vi "PicoScope2000AdvancedTriggerSettings.vi"(0 "handle in":i16, 2 "Pulse Width Qualifier Conditions":T4 {"Condition Logic" items=["AND", "OR", "XOR"]}, 3 "Pulse Width Qualifier Settings":T3 {"Pulse Width Type" items=["None", "Less Than", "Greater Than", "In Range", "Out of Range"]; "Direction" items=["Rising", "Falling"]}, 5 "error in":errorcluster, 6 "Trigger Conditions":T1 {"PWQ" items=["Don't Care", "True", "False"]; "Ext" items=["Don't Care", "True", "False"]; "Channel D" items=["Don't Care", "True", "False"]; "Channel C" items=["Don't Care", "True", "False"]; "Channel B" items=["Don't Care", "True", "False"]; "Channel A" items=["Don't Care", "True", "False"]; "Condition Logic" items=["AND", "OR", "XOR"]}, 7 "Auto Trigger (ms)":i32, 8 "Channel A Trigger Properties":T2 {"Direction" items=["Above / Inside", "Below / Outside", "Rising / Enter", "Falling / Exit", "Rising or Falling / Enter or Exit", "Above Lower", "Below Lower", "Rising Lower", "Falling Lower", "Positive Runt", "Negative Runt"]; "Threshold Mode" items=["Level", "Window"]}, 9 "Trigger Delay":u32, 10 "Channel B Trigger Properties":T2 {"Direction" items=["Above / Inside", "Below / Outside", "Rising / Enter", "Falling / Exit", "Rising or Falling / Enter or Exit", "Above Lower", "Below Lower", "Rising Lower", "Falling Lower", "Positive Runt", "Negative Runt"]; "Threshold Mode" items=["Level", "Window"]}, 11 "preTriggerDelay":sgl, 12 "Ext. Trigger Properties":T2 {"Direction" items=["Above / Inside", "Below / Outside", "Rising / Enter", "Falling / Exit", "Rising or Falling / Enter or Exit", "Above Lower", "Below Lower", "Rising Lower", "Falling Lower", "Positive Runt", "Negative Runt"]; "Threshold Mode" items=["Level", "Window"]}) -> (14 "handle out":i16, 19 "error out":errorcluster)   [LabVIEW 2009]
doc: "This VI is an interface for the advanced trigger features of the oscilloscope (a simple trigger can be set using PicoScope2000Settings.vi, in which case it is not necessary to use this VI)."
uses:
  ps2000.dll
panel:
  in  "Channel D Trigger Properties":T2 {"Direction" items=["Above / Inside", "Below / Outside", "Rising / Enter", "Falling / Exit", "Rising or Falling / Enter or Exit", "Above Lower", "Below Lower", "Rising Lower", "Falling Lower", "Positive Runt", "Negative Runt"]; "Threshold Mode" items=["Level", "Window"]}
  in  "Channel C Trigger Properties":T2 {"Direction" items=["Above / Inside", "Below / Outside", "Rising / Enter", "Falling / Exit", "Rising or Falling / Enter or Exit", "Above Lower", "Below Lower", "Rising Lower", "Falling Lower", "Positive Runt", "Negative Runt"]; "Threshold Mode" items=["Level", "Window"]}
  # "For Condition Logic Suggested settings;\nFor AND, XOR logic-(parallel triggers)\nUse level-type triggers (Level or Inside/outside Window Triggers)\n\nFor OR logic- (single channel)\nUse edge types (e.g. rising, falling, entering window)"
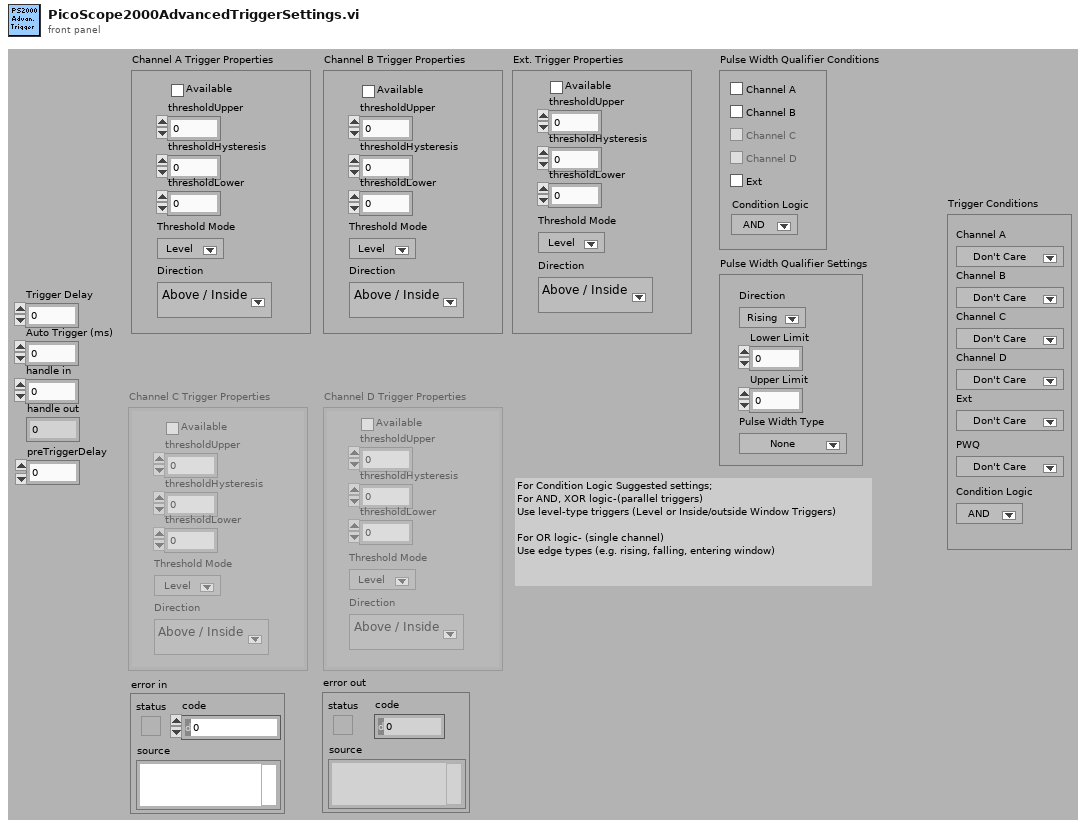
[diagram p1: front panel]
types:
  T1 = cluster{"Channel A":u16, "Channel B":u16, "Channel C":u16, "Channel D":u16, "Ext":u16, "PWQ":u16, "Condition Logic":u16}
  T2 = cluster{"thresholdUpper":i16, "thresholdHysteresis":u16, "thresholdLower":i16, "Threshold Mode":i32, "Direction":i32, "Available":bool}
  T3 = cluster{"Direction":u32, "Lower Limit":u32, "Upper Limit":u32, "Pulse Width Type":u32}
  T4 = cluster{"Channel A":bool, "Channel B":bool, "Channel C":bool, "Channel D":bool, "Condition Logic":u16, "Ext":bool}
  T5 = cluster{"thresholdUpper":i16, "thresholdHysteresis":u16, "thresholdLower":i16, "Threshold Mode":i32, "Direction":i32, "Available":bool}[]
  T6 = cluster{"[0]":u32, "[1]":u32, "[2]":u32, "[3]":u32, "[4]":u32, "[5]":u32, "[6]":u32, "[7]":u32, "[8]":u32}
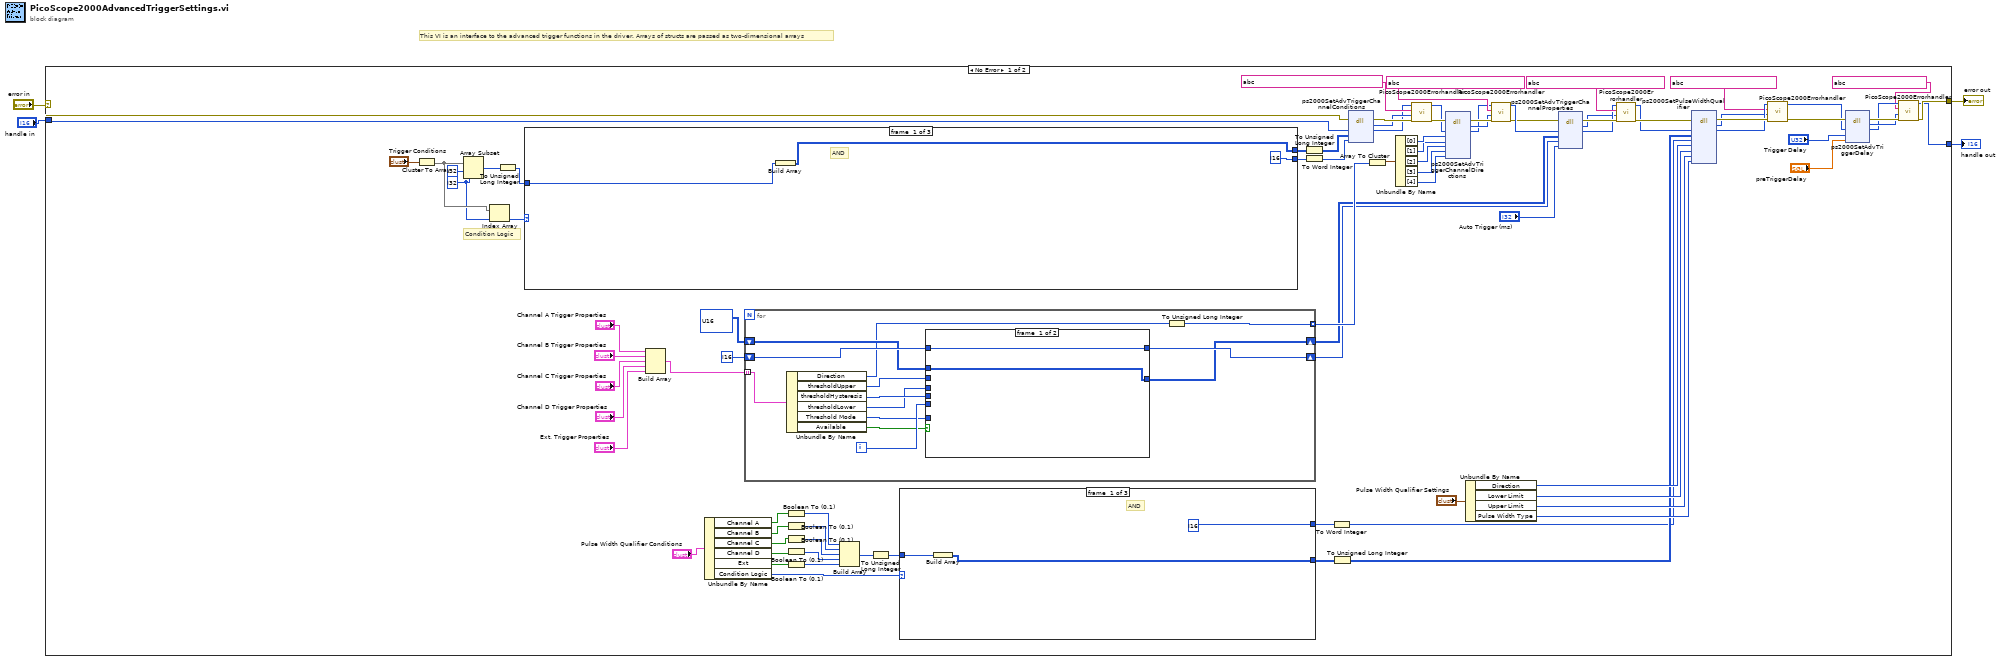
[diagram p0: block diagram]
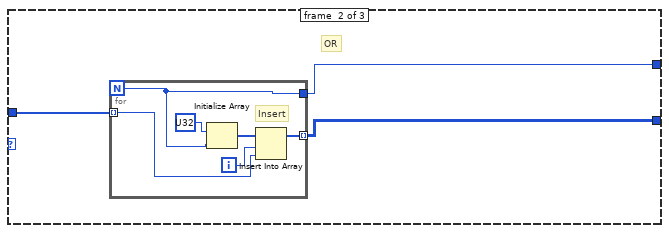
[diagram p2: hidden frame]
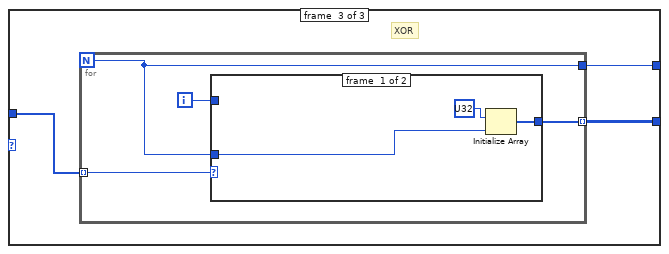
[diagram p3: hidden frame]
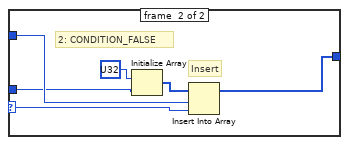
[diagram p4: hidden frame]
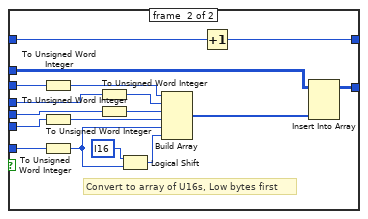
[diagram p5: hidden frame]
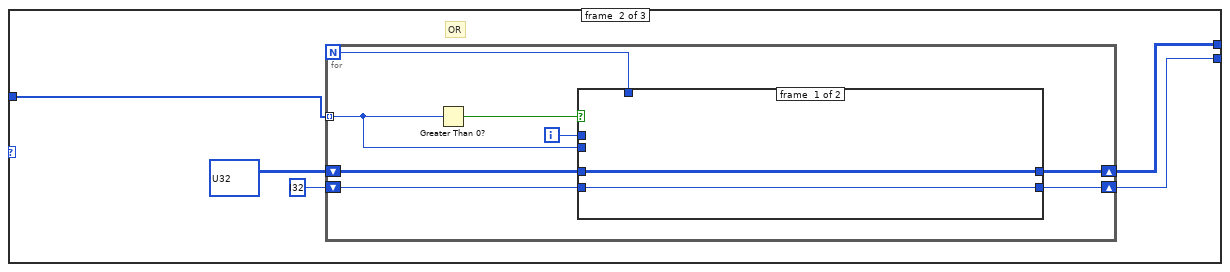
[diagram p6: hidden frame]
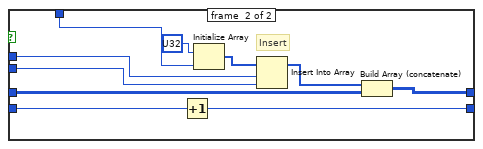
[diagram p7: hidden frame]
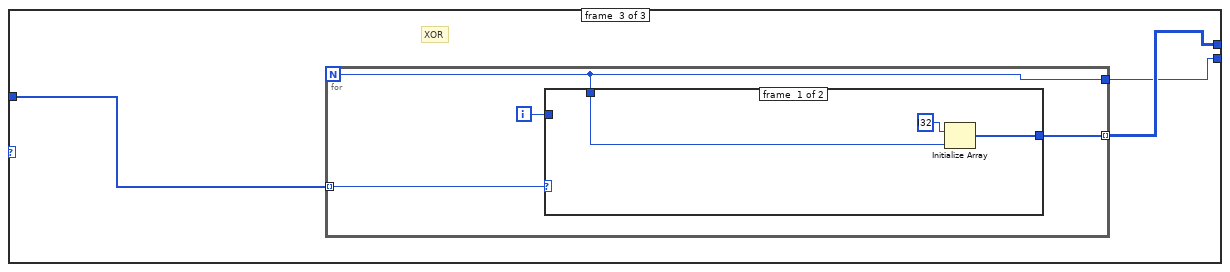
[diagram p8: hidden frame]
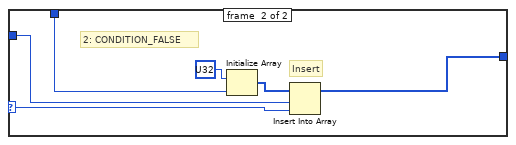
[diagram p9: hidden frame]
diagram:
  # "This VI is an interface to the advanced trigger functions in the driver. Arrays of structs are passed as two-dimensional arrays"
  n1 = case shown="No Error" "error in" {
    selector: "error in" -> [w67 w195]
    tunnel: "handle in" -> [w70 w196]
    tunnel: [w6 w196] -> w2
    tunnel: [w7 w195] -> w1
    frame #0 {
      w32 = i32 ? ("length")
      # "Condition Logic"
      n2 = Cluster To Array(cluster="Trigger Conditions") -> (array=w33:u16[])
      n3 = Array Subset(array=w33, index=i32 ?, length=w32) -> (w35:u16[])
      n4 = Index Array(array=w33, index=w32) -> (element=w34:u16)
      n5 = To Unsigned Long Integer(number=w35) -> (unsigned 32bit integer=w53:u32[])
      n6 = case shown="2" w34 {
        tunnel: [w153 w158 w181] -> w61
        tunnel: [i16 ? w154 w179] -> w52
        tunnel: w53 -> [w151 w155 w180]
        frame #0 {
          # "AND"
          n7 = Build Array(w151) -> (w153:u32[][])
        }
        frame #1 {
          # "OR"
          n8 = for {
            N -> [w159]
            tunnel: w155 -> [w163] mode=indexing
            shift-right: [w162] -> w158
            shift-left: u32[][] ? -> [w166]
            shift-right: [w160] -> w154
            shift-left: i32 ? -> [w161]
            i -> [w165]
            n9 = Greater Than 0?(x=w163) -> (x > 0?=w164:bool)
            n10 = case shown="True" w164 {
              tunnel: w166 -> [w168 w172]
              tunnel: w165 -> [_ w176]
              tunnel: w163 -> [_ w175]
              tunnel: [w168 w174] -> w162
              tunnel: w161 -> [w167 w171]
              tunnel: [w167 w170] -> w160
              tunnel: w159 -> [_ w169]
              frame #0 {
              }
              frame #1 {
                # "Insert"
                n11 = Increment(x=w171) -> (x+1=w170:i32)
                n12 = Initialize Array(u32 ? ("element"), w169) -> (w177:u32[])
                n13 = Insert Into Array(array=w177, index=w176, new element=w175) -> (w173:u32[])
                n14 = Build Array (concatenate)(w173, w172) -> (w174:u32[][])
              }
            }
          }
        }
        frame #2 {
          # "XOR"
          n15 = for {
            N -> [w182]
            tunnel: w180 -> [w183] mode=indexing
            tunnel: [w185] -> w181 mode=indexing
            tunnel: [w182] -> w179
            i -> [w184]
            n16 = case shown="1" w183 {
              selector: w183 -> [_ w191]
              tunnel: [w187 w192] -> w185
              tunnel: w184 -> [_ w190]
              tunnel: w182 -> [w186 w189]
              frame #0 {
                n17 = Initialize Array(i32 ? ("element"), w186) -> (w187:i32[])
              }
              frame #1 {
                # "2: CONDITION_FALSE"
                # "Insert"
                n18 = Initialize Array(u32 ? ("element"), w189) -> (w193:u32[])
                n19 = Insert Into Array(array=w193, index=w190, new element=w191) -> (w192:u32[])
              }
            }
          }
        }
      }
      n20 = Build Array("Channel A Trigger Properties", "Channel B Trigger Properties", "Channel C Trigger Properties", "Channel D Trigger Properties", "Ext. Trigger Properties") -> (w89:T5)
      n21 = Unbundle By Name("Pulse Width Qualifier Conditions") -> ("Channel A"=w41:bool, "Channel B"=w42:bool, "Channel C"=w43:bool, "Channel D"=w44:bool, "Ext"=w45:bool, "Condition Logic"=w40:u16)
      n22 = for {
        tunnel: w89 -> [w128] mode=indexing
        tunnel: [w121] -> w88 mode=indexing
        shift-right: [w126] -> w65
        shift-left: i16 ? -> [w125]
        shift-right: [w123] -> w63
        shift-left: u16[][] ? -> [w124]
        i -> [w127]
        n23 = Unbundle By Name(w128) -> ("Direction"=w122:i32, "thresholdUpper"=w131:i16, "thresholdHysteresis"=w130:u16, "thresholdLower"=w129:i16, "Threshold Mode"=w119:i32, "Available"=w120:bool)
        n24 = case shown="True" w120 {
          tunnel: w131 -> [_ w145]
          tunnel: w130 -> [_ w144]
          tunnel: w129 -> [_ w143]
          tunnel: w119 -> [_ w135]
          tunnel: w127 -> [_ w142]
          tunnel: [w133 w150] -> w126
          tunnel: w125 -> [w133 w149]
          tunnel: [w132 w147] -> w123
          tunnel: w124 -> [w132 w146]
          frame #0 {
          }
          frame #1 {
            # "Convert to array of U16s, Low bytes first"
            n25 = To Unsigned Word Integer(number=w145) -> (unsigned 16bit integer=w141:u16)
            n26 = To Unsigned Word Integer(number=w142) -> (unsigned 16bit integer=w138:u16)
            n27 = To Unsigned Word Integer(number=w135) -> (unsigned 16bit integer=w134:u16)
            n28 = To Unsigned Word Integer(number=w143) -> (unsigned 16bit integer=w140:u16)
            n29 = To Unsigned Word Integer(number=w144) -> (unsigned 16bit integer=w139:u16)
            n30 = Logical Shift(y=i16 ?, x=w134) -> (x << y=w136:u16)
            n31 = Build Array(w141, w140, w139, w138, w134, w136) -> (w148:u16[])
            n32 = Increment(x=w149) -> (x+1=w150:i16)
            n33 = Insert Into Array(array=w146, new element=w148) -> (w147:u16[][])  [unwired: 2 in]
          }
        }
        n34 = To Unsigned Long Integer(number=w122) -> (unsigned 32bit integer=w121:u32)
      }
      n35 = Boolean To (0,1)(Boolean=w41) -> (0, 1=w50:i16)
      n36 = Boolean To (0,1)(Boolean=w42) -> (0, 1=w49:i16)
      n37 = Boolean To (0,1)(Boolean=w43) -> (0, 1=w48:i16)
      n38 = Boolean To (0,1)(Boolean=w44) -> (0, 1=w47:i16)
      n39 = Boolean To (0,1)(Boolean=w45) -> (0, 1=w46:i16)
      n40 = Build Array(w50, w49, w48, w47, w46) -> (w39:i16[])
      n41 = To Unsigned Long Integer(number=w39) -> (unsigned 32bit integer=w38:u32[])
      n42 = case shown="2" w40 {
        tunnel: [w93 w96 w105] -> w60
        tunnel: [i16 ? w95 w104] -> w54
        tunnel: w38 -> [w91 w94 w103]
        frame #0 {
          # "AND"
          n43 = Build Array(w91) -> (w93:u32[][])
        }
        frame #1 {
          # "OR"
          n44 = for {
            N -> [w97]
            tunnel: w94 -> [w99] mode=indexing
            tunnel: [w98] -> w96 mode=indexing
            tunnel: [w97] -> w95
            i -> [w100]
            # "Insert"
            n45 = Initialize Array(u32 ? ("element"), w97) -> (w101:u32[])
            n46 = Insert Into Array(array=w101, index=w100, new element=w99) -> (w98:u32[])
          }
        }
        frame #2 {
          # "XOR"
          n47 = for {
            N -> [w106]
            tunnel: w103 -> [w109] mode=indexing
            tunnel: [w107] -> w105 mode=indexing
            tunnel: [w106] -> w104
            i -> [w108]
            n48 = case shown="1" w109 {
              selector: w109 -> [_ w115]
              tunnel: [w111 w116] -> w107
              tunnel: w108 -> [_ w114]
              tunnel: w106 -> [w110 w113]
              frame #0 {
                n49 = Initialize Array(u32 ? ("element"), w110) -> (w111:u32[])
              }
              frame #1 {
                # "2: CONDITION_FALSE"
                # "Insert"
                n50 = Initialize Array(u32 ? ("element"), w113) -> (w117:u32[])
                n51 = Insert Into Array(array=w117, index=w114, new element=w115) -> (w116:u32[])
              }
            }
          }
        }
      }
      n52 = To Unsigned Long Integer(number=w61) -> (unsigned 32bit integer=w62:u32[][])
      n53 = To Word Integer(number=w52) -> (16bit integer=w51:i16)
      n54 = To Word Integer(number=w54) -> (16bit integer=w55:i16)
      n55 = To Unsigned Long Integer(number=w60) -> (unsigned 32bit integer=w59:u32[][])
      n56 = dll-call lib="ps2000.dll" fn="ps2000SetAdvTriggerChannelConditions" ("ps3000.dll:_ps3000_open_unit@0")(error in=w67, "handle"=w70, "conditions"=w62, "nConditions"=w51) -> (error out=w69:errorcluster, "return"=w31:i16, "handle"=w30:i16)  [unwired: 4 in, 1 out]
      n57 = Array To Cluster(array=w88) -> (cluster=w87:T6)
      n58 = Unbundle By Name(w87) -> ("[0]"=w86:u32, "[1]"=w85:u32, "[2]"=w84:u32, "[3]"=w83:u32, "[4]"=w82:u32)
      n59 = call "PicoScope2000Errorhandler.vi"("Handle in"=w30, "API function"=string ? ("source"), "Return"=w31, "error in (no error)"=w69) -> ("Handle out"=w29:i16, "error out"=w58:errorcluster)  [unwired: 5 in]
      n60 = dll-call lib="ps2000.dll" fn="ps2000SetAdvTriggerChannelDirections" ("ps3000.dll:_ps3000_open_unit@0")(error in=w58, "handle"=w29, "channelA"=w86, "channelB"=w85, "channelC"=w84, "channelD"=w83, "ext"=w82) -> (error out=w28:errorcluster, "return"=w27:i16, "handle"=w25:i16)  [unwired: 7 in, 1 out]
      n61 = Unbundle By Name("Pulse Width Qualifier Settings") -> ("Direction"=w78:u32, "Lower Limit"=w77:u32, "Upper Limit"=w76:u32, "Pulse Width Type"=w75:u32)
      n62 = call "PicoScope2000Errorhandler.vi"("Handle in"=w25, "API function"=string ? ("source"), "Return"=w27, "error in (no error)"=w28) -> ("Handle out"=w24:i16, "error out"=w23:errorcluster)  [unwired: 5 in]
      n63 = dll-call lib="ps2000.dll" fn="ps2000SetAdvTriggerChannelProperties" ("ps3000.dll:_ps3000_open_unit@0")(error in=w23, "handle"=w24, "channelProperties"=w63, "nChannelProperties"=w65, "autoTriggerMilliseconds"="Auto Trigger (ms)") -> (error out=w22:errorcluster, "return"=w12:i16, "handle"=w13:i16)  [unwired: 5 in, 1 out]
      n64 = call "PicoScope2000Errorhandler.vi"("Handle in"=w13, "API function"=string ? ("source"), "Return"=w12, "error in (no error)"=w22) -> ("Handle out"=w11:i16, "error out"=w21:errorcluster)  [unwired: 5 in]
      n65 = dll-call lib="ps2000.dll" fn="ps2000SetPulseWidthQualifier" ("ps3000.dll:_ps3000_open_unit@0")(error in=w21, "handle"=w11, "conditions"=w59, "nConditions"=w55, "direction"=w78, "lower"=w77, "upper"=w76, "type"=w75) -> (error out=w20:errorcluster, "return"=w16:i16, "handle"=w17:i16)  [unwired: 8 in, 1 out]
      n66 = call "PicoScope2000Errorhandler.vi"("Handle in"=w17, "API function"=string ? ("source"), "Return"=w16, "error in (no error)"=w20) -> ("Handle out"=w18:i16, "error out"=w19:errorcluster)  [unwired: 5 in]
      n67 = dll-call lib="ps2000.dll" fn="ps2000SetAdvTriggerDelay" ("ps3000.dll:_ps3000_open_unit@0")(error in=w19, "handle"=w18, "delay"="Trigger Delay", "preTriggerDelay"="preTriggerDelay") -> (error out=w10:errorcluster, "return"=w9:i16, "handle"=w8:i16)  [unwired: 4 in, 1 out]
      n68 = call "PicoScope2000Errorhandler.vi"("Handle in"=w8, "API function"=string ? ("source"), "Return"=w9, "error in (no error)"=w10) -> ("Handle out"=w6:i16, "error out"=w7:errorcluster)  [unwired: 5 in]
    }
    frame #1 {
    }
  }
  "handle out" <- w2
  "error out" <- w1
